vi "Build VIH Deploy - Save Project to Prev Version.vi"(8 "error in":errorcluster, 9 "LV Version":string(combo)="14.0", 10 "Project file":path, 11 "Target Dir":path) -> (0 "error out":errorcluster, 3 "dup Target Dir":path)   [LabVIEW 2014]
doc: "::: VI Helpeks :::\nCopyright (c) 2000-2026 Konstantin Shifershteyn. All rights reserved."
panel:
  # "VI Helpeks\nCopyright (c) 2012-2026 Konstantin Shifershteyn"
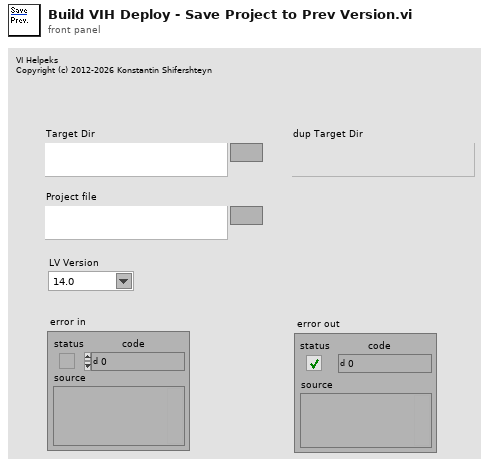
[diagram p1: front panel]
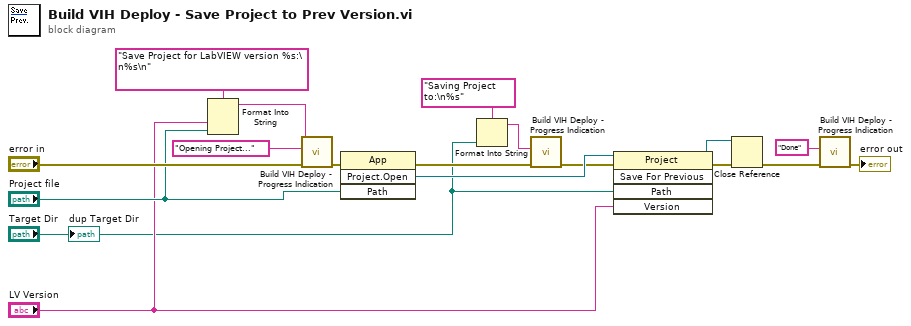
[diagram p0: block diagram]
diagram:
  n1 = Format Into String(format string="Save Project for LabVIEW version %s:\n%s\n", "LV Version", "Project file") -> (resulting string=w11:string)  [unwired: 2 in, 1 out]
  n2 = call "Build VIH Deploy - Progress Indication.vi"("error in"="error in", "message 2"="Opening Project...", "message 1"=w11) -> ("error out"=w4:errorcluster)  [unwired: 8 in]
  n3 = invoke class="App" method="Project.Open"(error in=w4, "Path"="Project file") -> (error out=w7:errorcluster, "Project:Open"=w16:refnum<vi>)  [unwired: 2 in, 2 out]
  n4 = Format Into String(format string="Saving Project to:\n%s", "Target Dir") -> (resulting string=w3:string)  [unwired: 2 in, 1 out]
  n5 = call "Build VIH Deploy - Progress Indication.vi"("error in"=w7, "message 2"=w3) -> ("error out"=w6:errorcluster)  [unwired: 9 in]
  n6 = invoke class="Project" method="Save For Previous"(reference=w16, error in=w6, "Path"="Target Dir", "Version"="LV Version") -> (reference out=w17:refnum<vi>, error out=w18:errorcluster)  [unwired: 1 in, 3 out]
  n7 = Close Reference(reference=w17, error in (no error)=w18) -> (error out=w14:errorcluster)
  n8 = call "Build VIH Deploy - Progress Indication.vi"("error in"=w14, "message 2"="Done") -> ("error out"=→"error out":errorcluster)  [unwired: 9 in]
  "dup Target Dir" <- "Target Dir"
